vi "Run Top Level.vi"(6 "Run/Open (T = Run)":bool=TRUE, 8 "error in":errorcluster, 9 "Alias":string, 10 "Project Reference":refnum<vi>) -> (0 "error out":errorcluster)   [LabVIEW 2020]
doc: "Run the top level VI in the project."
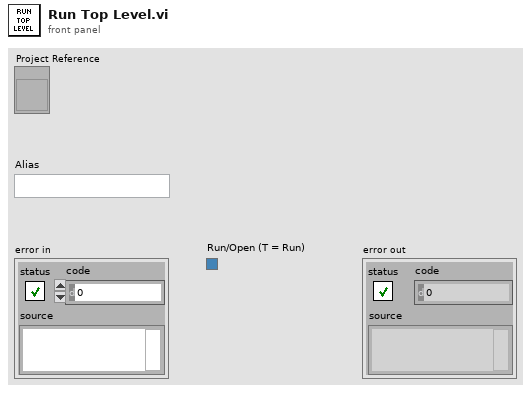
[diagram p1: front panel]
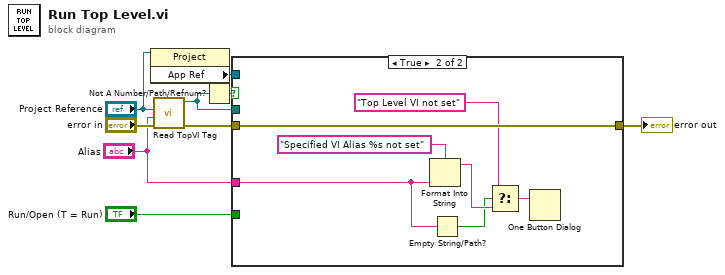
[diagram p0: block diagram]
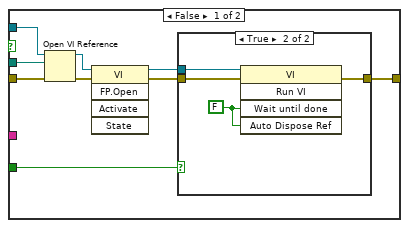
[diagram p2: hidden frame]
diagram:
  n1 = property class="Project"(reference="Project Reference") -> ("App Ref"=w3:refnum<vi>)  [unwired: 1 in, 2 out]
  n2 = call "Read TopVI Tag.vi"("error in"="error in", "Alias"="Alias", "Project Reference"="Project Reference") -> ("error out"=w7:errorcluster, "TopVI Path"=w6:path)  [unwired: 6 in, 1 out]
  n3 = Not A Number/Path/Refnum?(number/path/refnum=w6) -> (NaN/Path/Refnum?=w5:bool)
  n4 = case shown="True" w5 {
    tunnel: [w18 w30] -> w8
    tunnel: w7 -> [w17 w30]
    tunnel: w6 -> [w14 _]
    tunnel: w3 -> [w13 _]
    tunnel: "Run/Open (T = Run)" -> [w10 _]
    tunnel: "Alias" -> [_ w26]
    frame False {
      n5 = Open VI Reference(application reference (local)=w13, vi path=w14, error in (no error)=w17) -> (vi reference=w12:refnum<vi>, error out=w16:errorcluster)  [unwired: 3 in]
      n6 = invoke class="VI" method="FP.Open"(reference=w12, error in=w16) -> (reference out=w11:refnum<vi>, error out=w15:errorcluster)  [unwired: 3 in, 3 out]
      n7 = case shown="True" w10 {
        tunnel: [w19 w23] -> w18
        tunnel: w15 -> [w19 w22]
        tunnel: w11 -> [_ w20]
        frame False {
        }
        frame True {
          w21 = FALSE ("Auto Dispose Reference")
          n8 = invoke class="VI" method="Run VI"(reference=w20, error in=w22, "Wait until done"=w21, "Auto Dispose Ref"=w21) -> (error out=w23:errorcluster)  [unwired: 1 in, 4 out]
        }
      }
    }
    frame True {
      n9 = Format Into String(format string="Specified VI Alias %s not set" ("t"), w26) -> (resulting string=w28:string)  [unwired: 2 in, 1 out]
      n10 = Empty String/Path?(string/path=w26) -> (empty?=w25:bool)
      n11 = Select(t="Top Level VI not set", s=w25, f=w28) -> (s? t:f=w27:string)
      n12 = One Button Dialog(message=w27) -> ()  [unwired: 1 in, 1 out]
    }
  }
  "error out" <- w8
